vi "Begin.vi"(8 "error in":errorcluster) -> (0 "error out":errorcluster)   [LabVIEW 2016]
doc: "Called before other user functions, this VI is expected to open initial I/O refnums, load in file data, and do all program initialization. Notice that the <B>error out</B> terminal is simply used for data flow. Wiring it to other structures or subVIs ensures that this VI runs first."
uses:
  <vilib>/Rock Robotics/WPI/DriverStation/WPI_DriverStationRobotMode2.ctl
  <vilib>/Rock Robotics/SystemInterfaces/i2clib/i2c_bus.ctl
  Extra/TypeDefs/AutoMode_Type.ctl
  Extra/TypeDefs/DB/dbButtonDisplayNames_Type.ctl
  Extra/TypeDefs/DB/dbLEDDisplayNames_Type.ctl
  Extra/TypeDefs/DB/dbSliderDisplayNames_Type.ctl
  Extra/TypeDefs/DB/dbStringDisplayNames_Type.ctl
  Robot Global Data.vi
  <vilib>/Rock Robotics/Network Tables/NT Write String Array.vi
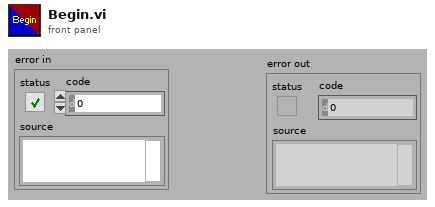
[diagram p1: front panel]
types:
  T1 = typedef "dbStringDisplayNames_Type.ctl" = enum16{"String 0", "String 1", "String 2", "String 3", "String 4", "String 5", "String 6", "String 7", "String 8", "String 9"}
  T2 = typedef "dbSliderDisplayNames_Type.ctl" = enum16{"MiddleAutoDist (in)", "SideAutoDist (in)", "AutoSpeed", "RailCenterOffset (in)"}
  T3 = typedef "dbLEDDisplayNames_Type.ctl" = enum16{"CATCH", "CATCH|", "CATCH||", "CATCH|||"}
  T4 = typedef "dbButtonDisplayNames_Type.ctl" = enum16{"CATCH", "CATCH|", "CATCH||", "CATCH|||"}
  T5 = typedef "AutoMode_Type.ctl" = enum16{"GearRight", "GearMiddle", "GearLeft", "Shoot&GearMiddle", "BaselineOnly"}
  T6 = typedef "i2c_bus.ctl" = enum16{"I2C On-Board", "I2C MXP", "Invalid"}
  T7 = typedef "WPI_DriverStationRobotMode2.ctl" = enum16{"Autonomous Disabled", "Autonomous Enabled", "Teleop Disabled", "Teleop Enabled", "Disconnected", "Finish", "Test Disabled", "Test Enabled", "Emergency Stopped"}
  T8 = typedef "WPI_I2CDevRef.ctl" = cluster{"DevStatus":errorcluster, "Device Address":u8, "Handle":i32, "I2C Bus":T6}
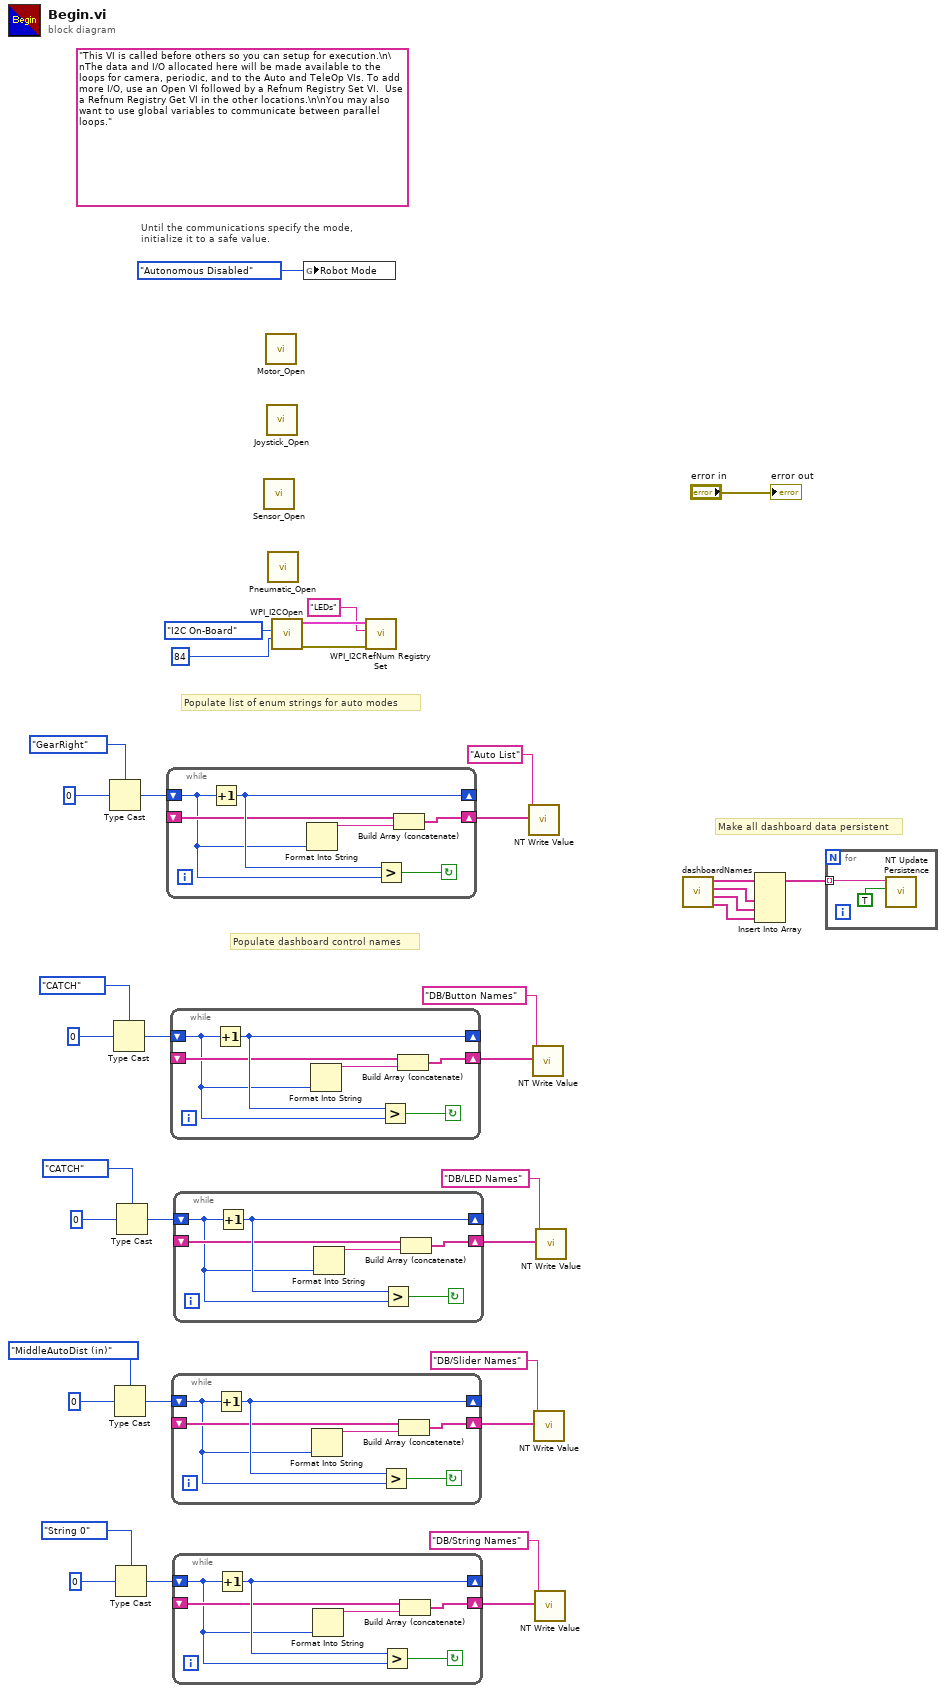
[diagram p0: block diagram]
diagram:
  (unwired) "This VI is called before others so you can setup for execution.\n\nThe data and I/O allocated here will be made available to the loops for camera, periodic, and to the Auto and TeleOp VIs. To add more I/O, use an Open VI followed by a Refnum Registry Set VI.  Use a Refnum Registry Get VI in the other locations.\n\nYou may also want to use global variables to communicate between parallel loops."
  # "Make all dashboard data persistent"
  # "Populate dashboard control names"
  # "Populate list of enum strings for auto modes"
  # "Until the communications specify the mode,\ninitialize it to a safe value."
  n1 = Type Cast(type=AutoMode_Type."GearRight" ("AutoMode"), x=0) -> (*(type *) &x=w27:T5)
  n2 = Type Cast(type=dbButtonDisplayNames_Type."CATCH" ("AutoMode"), x=0) -> (*(type *) &x=w24:T4)
  n3 = Type Cast(type=dbSliderDisplayNames_Type."MiddleAutoDist (in)" ("AutoMode"), x=0) -> (*(type *) &x=w14:T2)
  n4 = Type Cast(type=dbStringDisplayNames_Type."String 0" ("AutoMode"), x=0) -> (*(type *) &x=w7:T1)
  n5 = Type Cast(type=dbLEDDisplayNames_Type."CATCH" ("AutoMode"), x=0) -> (*(type *) &x=w17:T3)
  n6 = while {
    shift-right: [w42] -> _
    shift-left: w27 -> [w38]
    shift-right: [w40] -> w26
    shift-left: _ -> [w41]
    stop <- w43 continue-if-true
    n7 = Increment(x=w38) -> (x+1=w42:T5)
    n8 = Format Into String(w38) -> (resulting string=w39:string)  [unwired: 3 in, 1 out]
    n9 = Greater?(x=w42, y=w38) -> (0:w43:bool)
    n10 = Build Array (concatenate)(w41, w39) -> (w40:string[])
  }
  n11 = while {
    shift-right: [w48] -> _
    shift-left: w24 -> [w44]
    shift-right: [w46] -> w25
    shift-left: _ -> [w47]
    stop <- w49 continue-if-true
    n12 = Increment(x=w44) -> (x+1=w48:T4)
    n13 = Format Into String(w44) -> (resulting string=w45:string)  [unwired: 3 in, 1 out]
    n14 = Greater?(x=w48, y=w44) -> (0:w49:bool)
    n15 = Build Array (concatenate)(w47, w45) -> (w46:string[])
  }
  n16 = while {
    shift-right: [w54] -> _
    shift-left: w14 -> [w50]
    shift-right: [w52] -> w15
    shift-left: _ -> [w53]
    stop <- w55 continue-if-true
    n17 = Increment(x=w50) -> (x+1=w54:T2)
    n18 = Format Into String(w50) -> (resulting string=w51:string)  [unwired: 3 in, 1 out]
    n19 = Greater?(x=w54, y=w50) -> (0:w55:bool)
    n20 = Build Array (concatenate)(w53, w51) -> (w52:string[])
  }
  n21 = while {
    shift-right: [w60] -> _
    shift-left: w7 -> [w56]
    shift-right: [w58] -> w6
    shift-left: _ -> [w59]
    stop <- w61 continue-if-true
    n22 = Increment(x=w56) -> (x+1=w60:T1)
    n23 = Format Into String(w56) -> (resulting string=w57:string)  [unwired: 3 in, 1 out]
    n24 = Greater?(x=w60, y=w56) -> (0:w61:bool)
    n25 = Build Array (concatenate)(w59, w57) -> (w58:string[])
  }
  n26 = while {
    shift-right: [w66] -> _
    shift-left: w17 -> [w62]
    shift-right: [w64] -> w16
    shift-left: _ -> [w65]
    stop <- w67 continue-if-true
    n27 = Increment(x=w62) -> (x+1=w66:T3)
    n28 = Format Into String(w62) -> (resulting string=w63:string)  [unwired: 3 in, 1 out]
    n29 = Greater?(x=w66, y=w62) -> (0:w67:bool)
    n30 = Build Array (concatenate)(w65, w63) -> (w64:string[])
  }
  n31 = call "Sensor_Open.vi"() -> ()  [unwired: 12 in]
  n32 = call "Motor_Open.vi"() -> ()  [unwired: 12 in]
  n33 = call "Joystick_Open.vi"() -> ()  [unwired: 12 in]
  n34 = call "Pneumatic_Open.vi"() -> ()  [unwired: 12 in]
  n35 = call <vilib>:"WPI_I2COpen.vi"("Device Address"=u8 84, "I2C Bus"=i2c_bus."I2C On-Board") -> ("error out"=w33:errorcluster, "I2CDevRef"=w32:T8)  [unwired: 8 in]
  n36 = global write "Robot Global Data.vi" "Robot Mode"(WPI_DriverStationRobotMode2."Autonomous Disabled" ("Robot Mode")) -> ()
  n37 = call <vilib>:"WPI_I2CRefNum Registry Set.vi"("error in (no error)"=w33, "refnum name"="LEDs", "I2CDevRef"=w32) -> ()  [unwired: 7 in, 2 out]
  n38 = call-poly <vilib>:"NT Write Value.vi"("String Array"=w26, "Name"="Auto List") -> ()  [unwired: 9 in, 1 out]
  n39 = call-poly <vilib>:"NT Write Value.vi"("String Array"=w25, "Name"="DB/Button Names") -> ()  [unwired: 9 in, 1 out]
  n40 = call-poly <vilib>:"NT Write Value.vi"("String Array"=w15, "Name"="DB/Slider Names") -> ()  [unwired: 9 in, 1 out]
  n41 = call-poly <vilib>:"NT Write Value.vi"("String Array"=w6, "Name"="DB/String Names") -> ()  [unwired: 9 in, 1 out]
  n42 = call-poly <vilib>:"NT Write Value.vi"("String Array"=w16, "Name"="DB/LED Names") -> ()  [unwired: 9 in, 1 out]
  n43 = call "dashboardNames.vi"() -> ("String Names"=w1:string[], "Slider Names"=w2:string[], "LED Names"=w3:string[], "Button Names"=w5:string[])  [unwired: 8 in]
  n44 = Insert Into Array(array=w5, new element #1=w3, new element #2=w2, new element #3=w1) -> (w4:string[])  [unwired: 1 in]
  n45 = for {
    tunnel: w4 -> [w69] mode=indexing
    n46 = call <vilib>:"NT Update Persistence.vi"("Persistence"=TRUE, "Name"=w69) -> ()  [unwired: 9 in, 1 out]
  }
  "error out" <- "error in"
